vi "Initialize Stream Timing If Necessary.vi"(8 "error in (no error)":errorcluster, 11 "Modbus in":refnum<class "Modbus.lvclass">) -> (0 "error out":errorcluster, 3 "Modbus out":refnum<class "Modbus.lvclass">)   [LabVIEW 2026, in "Modbus.lvlib" / "Modbus.lvclass"]
uses:
  Modbus.lvclass
  Modbus.lvclass/Modbus.ctl
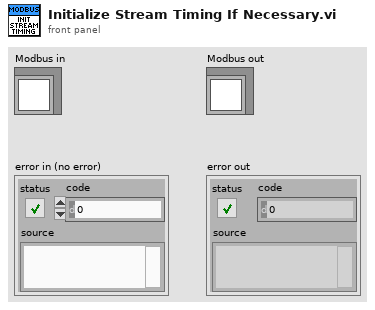
[diagram p1: front panel]
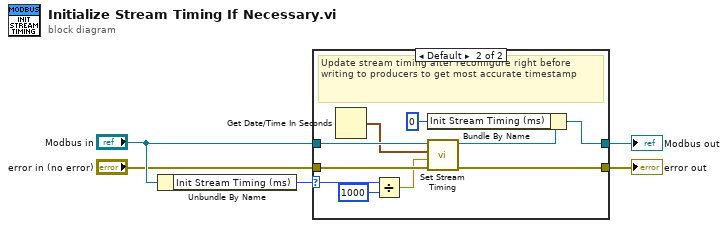
[diagram p0: block diagram]
diagram:
  n1 = Unbundle By Name("Modbus in") -> ("Init Stream Timing (ms)"=w1:i32)
  n2 = case shown="Default" w1 {
    selector: w1 -> [_ w11]
    tunnel: "Modbus in" -> [w7 w17]
    tunnel: [w6 w16] -> w4
    tunnel: "error in (no error)" -> [w6 w15]
    tunnel: [w7 w8] -> w2
    frame 0 {
    }
    frame Default {
      # "Update stream timing after reconfigure right before writing to producers to get most accurate timestamp"
      n3 = Get Date/Time In Seconds() -> (seconds since 1Jan1904=w13:timestamp)
      n4 = Divide(x=w11, y=1000) -> (x/y=w14:dbl)
      n5 = call-dynamic "Set Stream Timing.vi"("error in (no error)"=w15, "dt(sec)"=w14, "Start Time"=w13, "Plugin in"=w17) -> ("error out"=w16:errorcluster, "Plugin out"=w10:refnum<class "Modbus.lvclass">)  [unwired: 6 in]
      n6 = Bundle By Name(cluster=w10, "Init Stream Timing (ms)"=0) -> (w8:refnum<class "Modbus.lvclass">)
    }
  }
  "error out" <- w4
  "Modbus out" <- w2
